vi "Start_Time.vi"(8 "error in (no error)":errorcluster) -> (0 "error in (no error) 3":errorcluster)   [LabVIEW 2021]
uses:
  Template/Main_VI/Control/Ini.ctl
panel:
  out "Time stamp":string
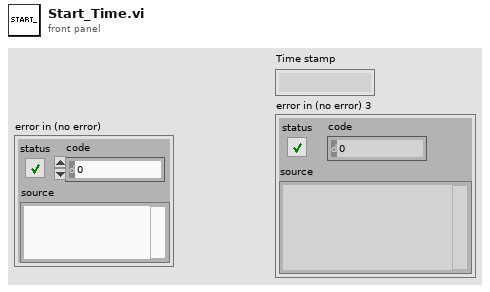
[diagram p1: front panel]
types:
  T1 = typedef "Ini.ctl" = enum16{"Write", "Read"}
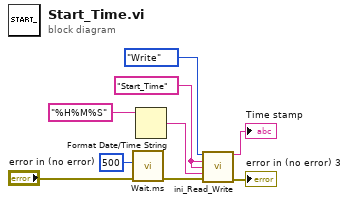
[diagram p0: block diagram]
diagram:
  w6 = "Start_Time" ("Write Section")
  n1 = call "Wait.ms.vi"("error in"="error in (no error)", "milliseconds to wait"=u32 500) -> ("error out"=w2:errorcluster)  [unwired: 9 in]
  n2 = Format Date/Time String(time format string (%c)="%H%M%S") -> (date/time string=w5:string)  [unwired: 2 in]
  n3 = call "ini_Read_Write.vi"(0:Ini."Write", "Write Section"=w6, "Write key"=w6, "Write"=w5, "error in (no error) 2"=w2) -> ("value"=→"Time stamp":string, "error in (no error) 3"=→"error in (no error) 3":errorcluster)  [unwired: 9 in]
